vi "Find Center.vi"(5 "Position":i32, 7 "Tray Number":dbl format="%#_13g", 8 "Assembly Type":string, 9 "XYZTheta":dbl[](array[numeric]), 11 "Gantry In":refnum<k24>) -> (0 "Pedestal Height":dbl[](array[numeric]), 1 "XYZTheta Centers":dbl[][](array[numeric]), 3 "Gantry Out":refnum<k24>)   [LabVIEW 2021, in "Assembly Tray.lvclass"]
uses:
  Assembly Tray.lvclass
  Find Tray.ctl
  Controller/Camera/Machine Vision.ctl
  C:/Program Files (x86)/Aerotech/A3200/LabVIEW/2010/Bin/Aerotech.A3200.dll
  Program Files (x86)/Aerotech/A3200/LabVIEW/2010/Bin/Aerotech.A3200.dll
  Controller/Camera/Image processing.ctl
  Controller/Camera/Camera settings.ctl
  Controller/Camera/Material.ctl
  Controller/Camera/Camera.lvclass
  Controller/Motion/A3200/A3200.lvclass
  Controller/Motion/Motion.lvclass
panel:
  out "Current Z High Speed":dbl
  out "Current XY High Speed":dbl
  out "current Z low speed":dbl
  out "current XY speed":dbl
  in  "Z high":dbl=12.5
  in  "XY high":dbl=50.0
  in  "Z low":dbl=0.05
  in  "XY low":dbl=0.1
  out "Low Speed":bool
  out "X":bool
  out "Y":bool
  out "Z":bool
  out "High Speed":bool
  out "Move by":dbl[](array[numeric])
  in  "Autofiducial (Beta)":bool
  in  "Focus step size":dbl format="%#_13g"
  in  "number of focus steps":i32
  out "Average Strength":dbl
  in  "Focus":bool
  in  "Material":T1
  in  "Camera settings":T2={"Gamma"=1.6, "Gain"=0, "Sharpness"=0, "Contrast"=0.0, "Exposure"=0.0078125} {"Exposure" min=0.000244140625 max=0.5 scale=0.0002..0.5; "Contrast" min=0.0 max=1.0 scale=0.001..1.0; "Sharpness" min=0 max=2 step=1 scale=0.0..2.0; "Gain" min=0 max=100 step=1 scale=0.1..100.0; "Gamma" min=0.01 max=10.0 scale=0.01..10.0}
  in  "Image processing":T3={"Brightness"=128.0, "Contrast"=45.0, "Gamma"=1.0471123} {"Brightness" scale=0.0..400.0; "Contrast" scale=0.0..90.0; "Gamma" scale=0.005..5.0}
  in  "Override presets":bool
  out "Both fiducials recorded":bool
  in  "Machine Vision":T4
  out "Right Fiducial":dbl[](array[numeric]) format="%.6g"
  out "Left Fiducial":dbl[](array[numeric]) format="%.6g"
  out "Gantry":dbl[](array[numeric]) format="%.6g"
  out "Sum":dbl[](array[numeric]) format="%.6g"
  out "Camera":dbl[](array[numeric]) format="%.6g"
  in  "Carrier Tray":T5
  out "Image":T6(plugin-control)
  out "Center":dbl[](array[numeric]) format="%.6g"
  in  "Position Number":i16
  in  "Go to Center":bool
  in  "Calculate":bool
  in  "Record Bottom":bool
  in  "Record Top":bool
  in  "Go to Bottom Fiducial":bool
  in  "Go to Top Fiducial":bool
  in  "Joystick":bool
  in  "Stop":bool
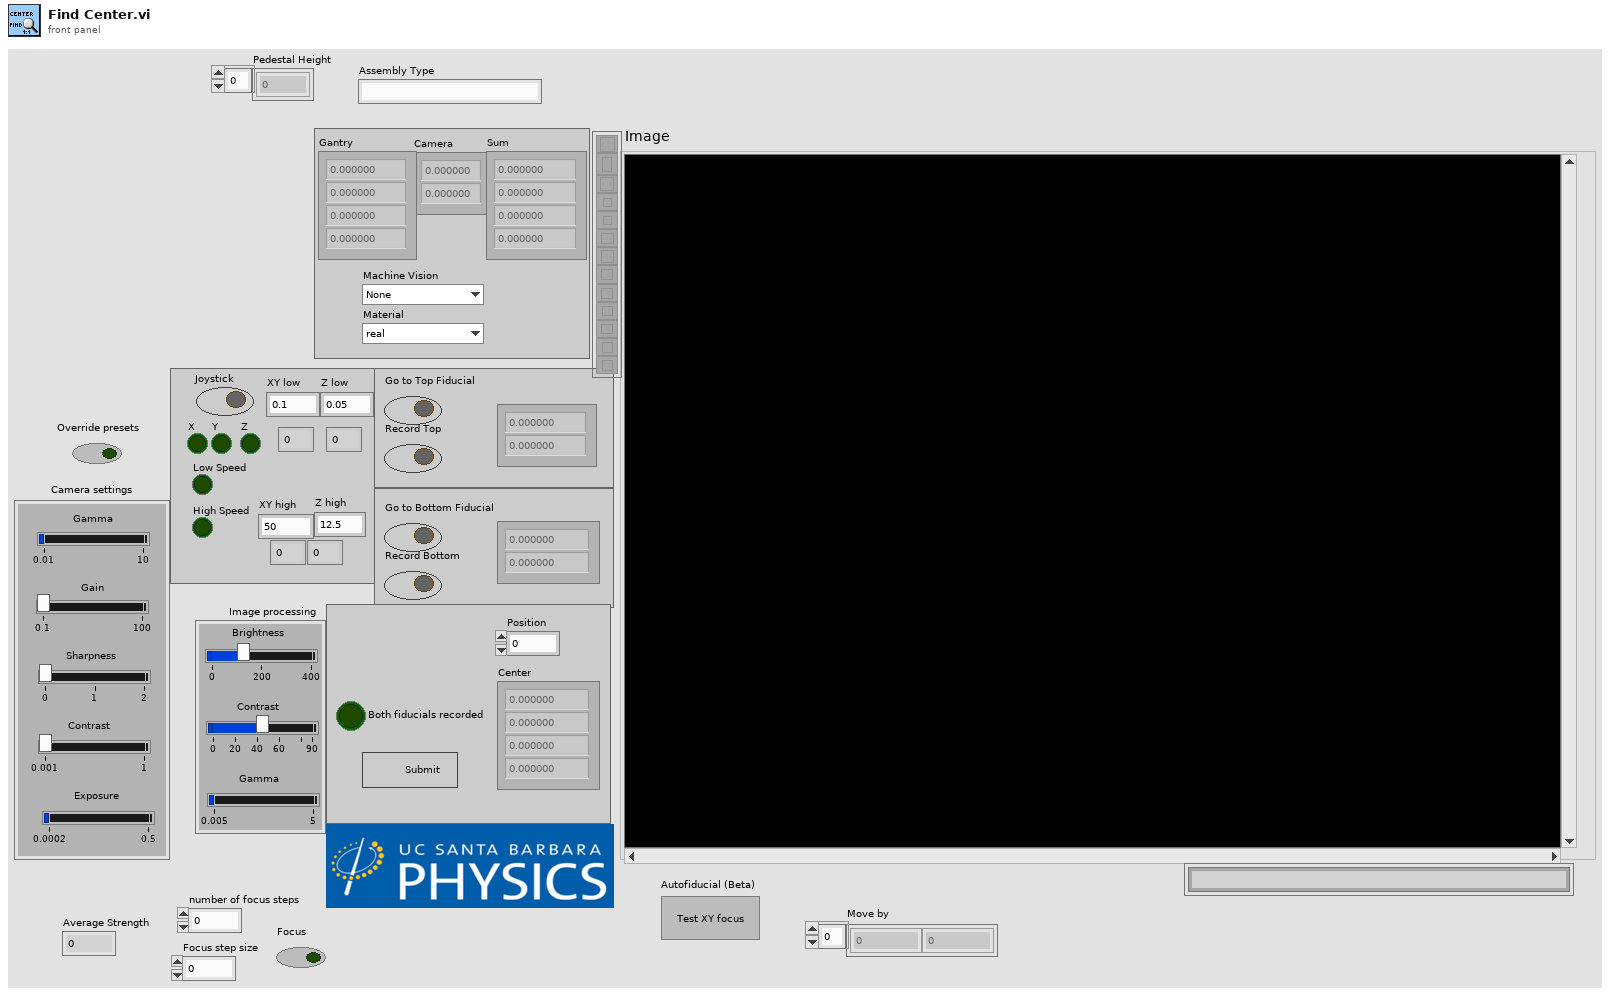
[diagram p1: front panel]
types:
  T1 = typedef "Camera.lvclass/Material.ctl" = enum16{"real", "dummy", "PETG"}
  T2 = typedef "Camera.lvclass/Camera settings.ctl" = cluster{"Gamma":dbl, "Gain":i64, "Sharpness":i64, "Contrast":dbl, "Exposure":dbl}
  T3 = typedef "Camera.lvclass/Image processing.ctl" = cluster{"Brightness":sgl, "Contrast":sgl, "Gamma":sgl}
  T4 = typedef "Camera.lvclass/Machine Vision.ctl" = enum16{"None", "Tray Fiducials", "Sensor Fiducials", "HPK Silicon", "Partial Hexaboard", "Partial Hexaboard Test", "100um dot", "Hexaboard", "Corner (TL, BR)", "Corner (BL, TR)", "V3 Sensor Cross", "V3 Sensor Circle", "test"}
  T5 = typedef "Assembly Tray.lvclass/Find Tray.ctl" = cluster{"Gantry Fiducials":dbl[], "Relative Coordinates":dbl[][], "Camera Fiducials":dbl[][], "XYZTheta Centers":dbl[][], "Workspace Center":dbl[], "Syringe Relative Coordinates":dbl[], "Gantry Region":dbl, "Fiducials":path, "New Fiducials":dbl[][], "Past Fiducials":dbl[][], "XYZTheta":dbl[], "Pedestal Height":dbl[]}
  T6 = typedef "IMAQ Image.ctl" = refnum<image>
  T7 = typedef "File Paths.ctl" = cluster{"Glue Pattern Folder":path, "Carrier Tray Folder":path, "Pick Up Tool Fixture Folder":path, "Components Folder":path, "Bellows Tool Offset.txt":path, "Pick Up Tool Offset.txt":path, "Dispense Tip Offset.txt":path, "Log Files":path, "Gantry Assembly Map.txt":path, "Syringe and offset map.txt":path, "Controllers Folder":path, "Local dbase config":path}
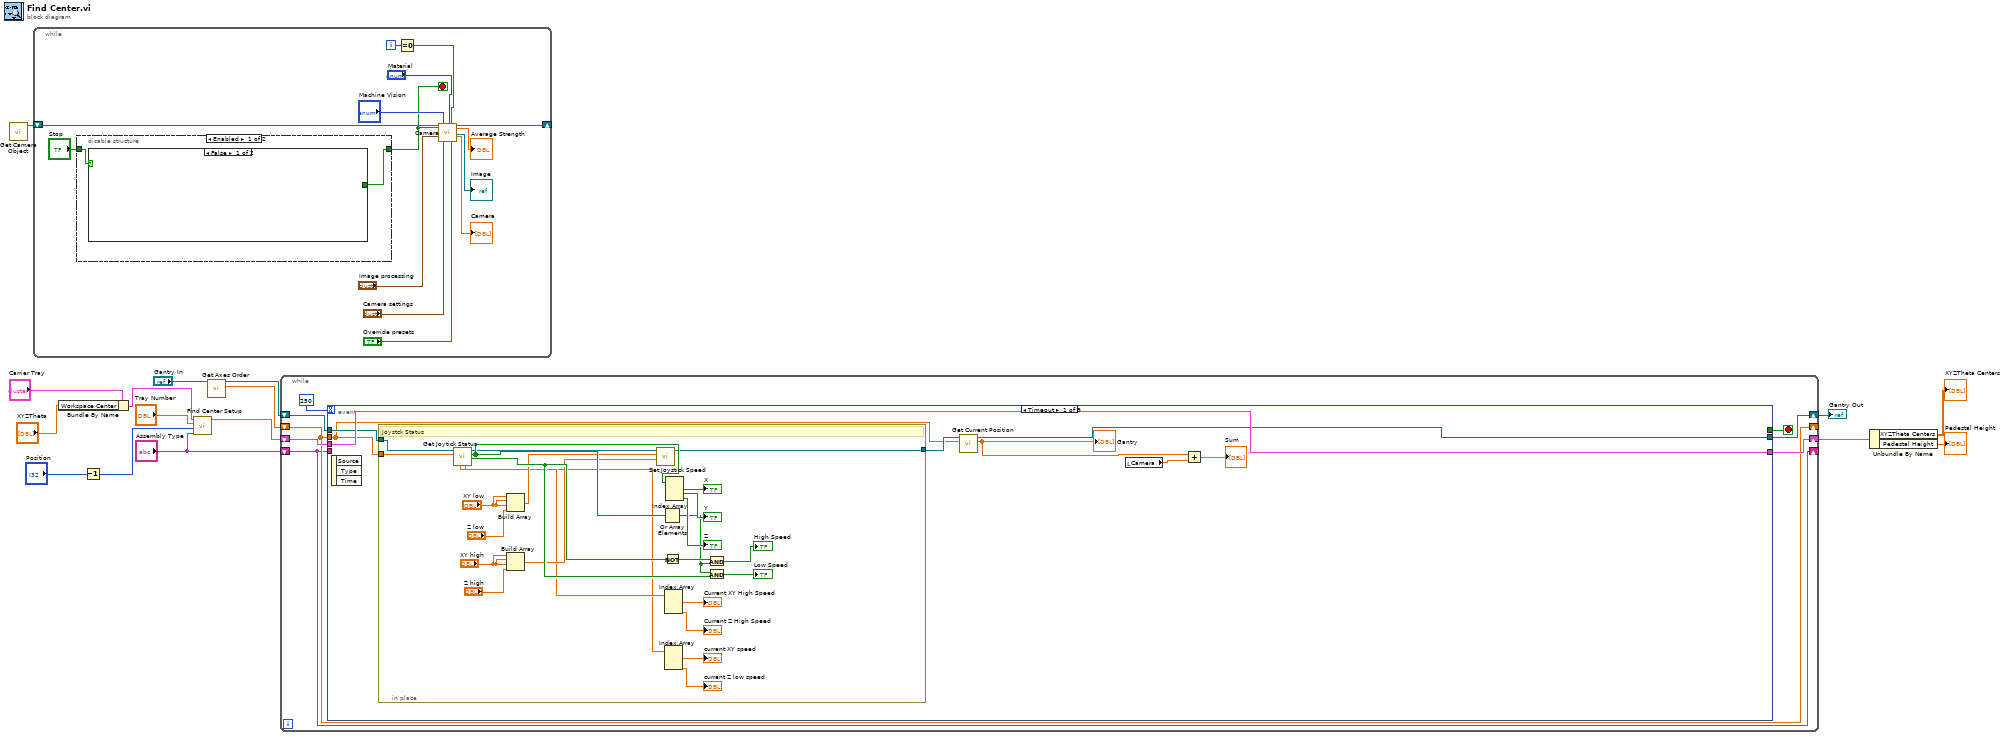
[diagram p0: block diagram]
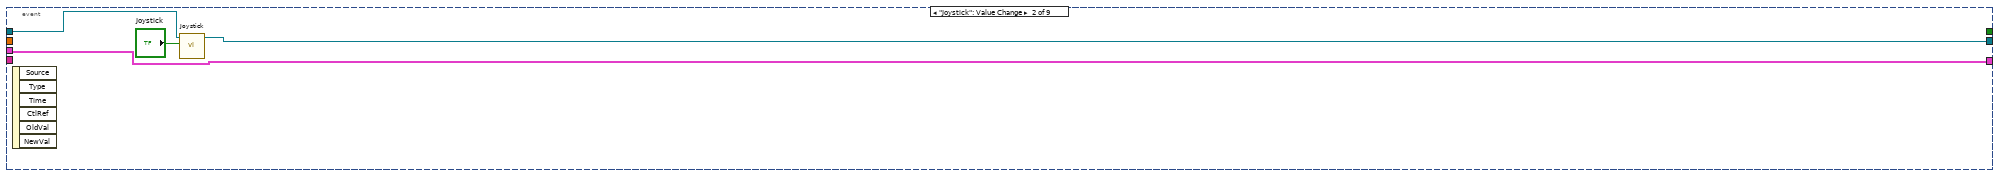
[diagram p2: hidden frame]
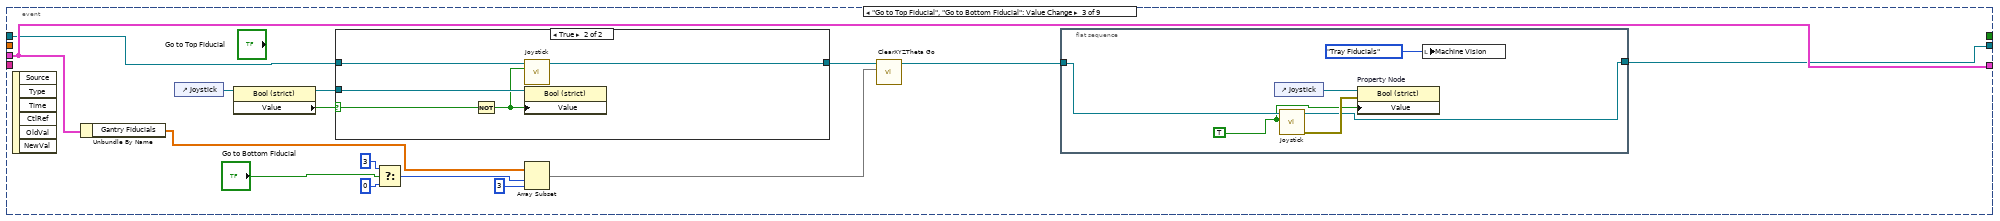
[diagram p3: hidden frame]
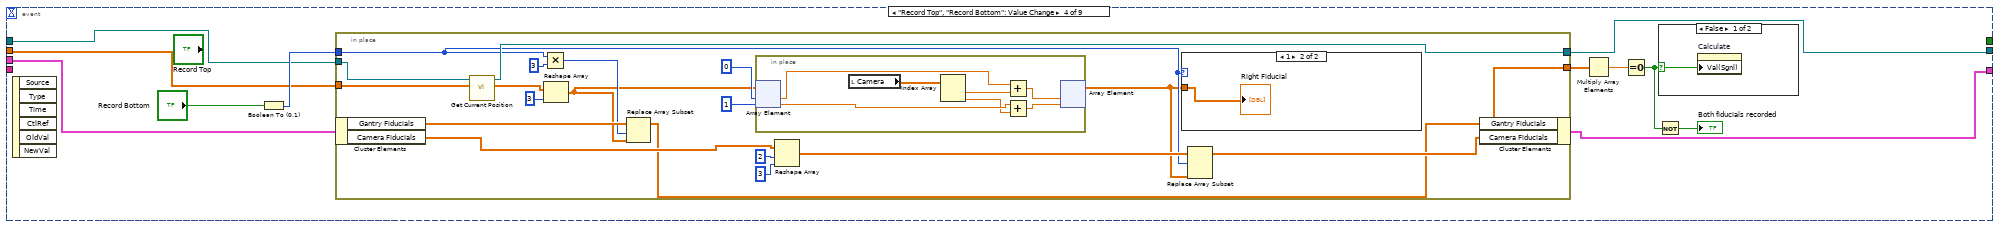
[diagram p5: hidden frame]
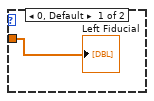
[diagram p7: hidden frame]
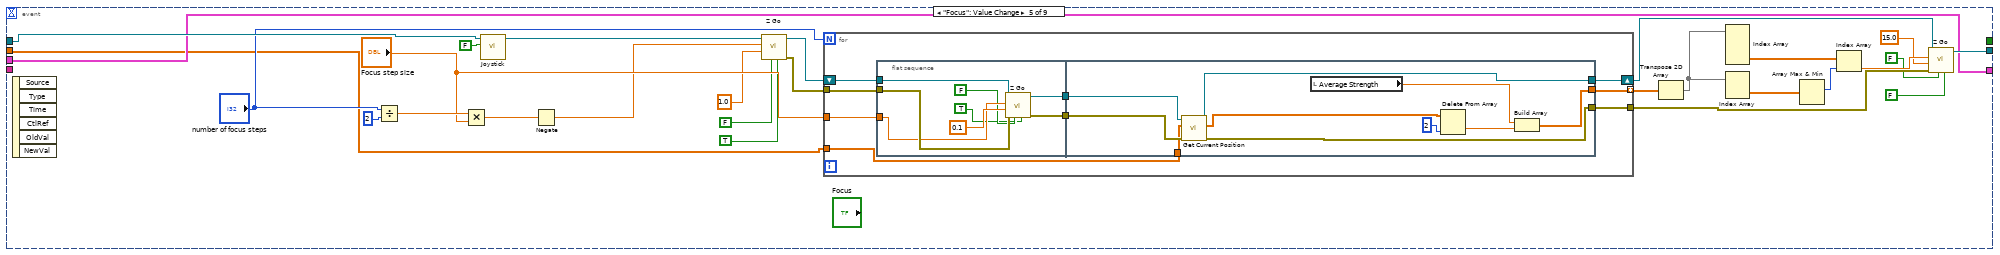
[diagram p8: hidden frame]
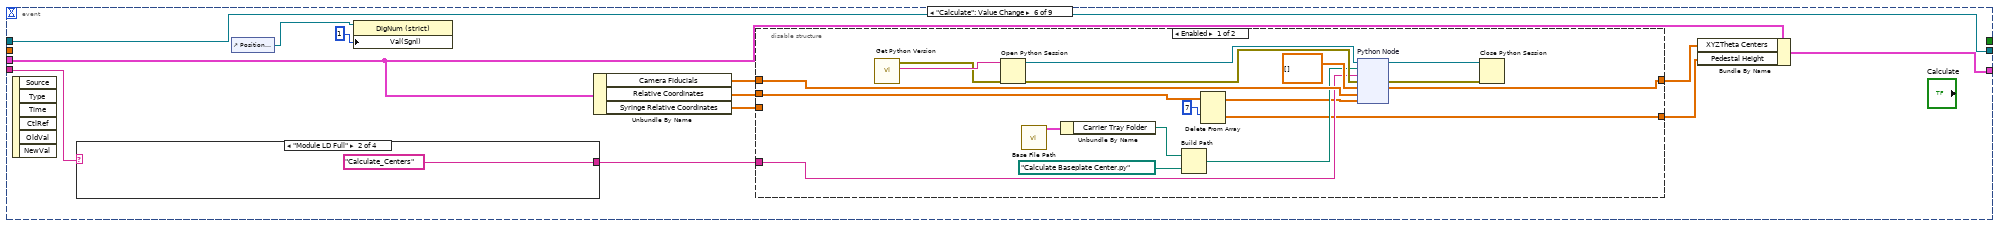
[diagram p9: hidden frame]
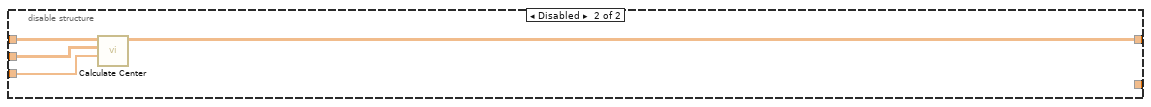
[diagram p10: hidden frame]
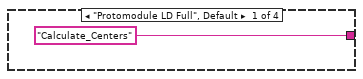
[diagram p11: hidden frame]
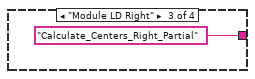
[diagram p12: hidden frame]
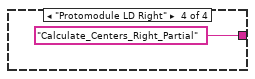
[diagram p13: hidden frame]
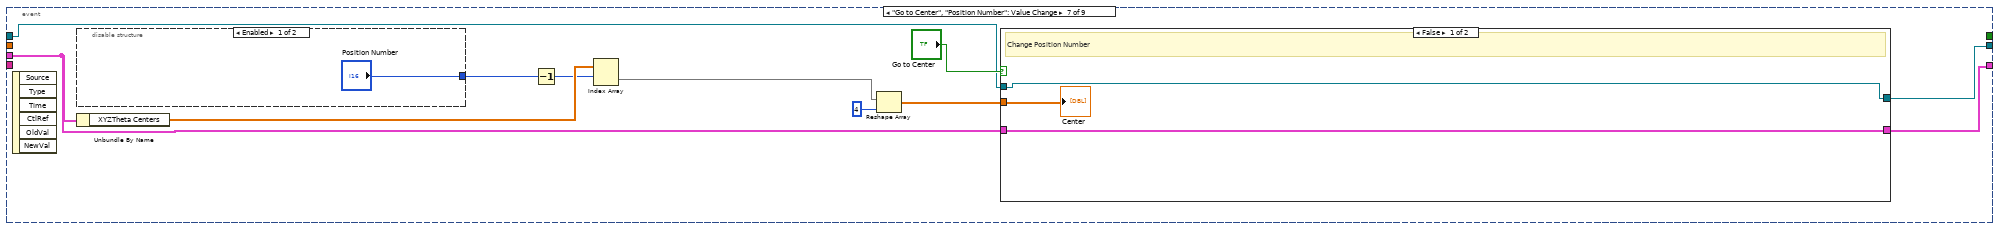
[diagram p14: hidden frame]
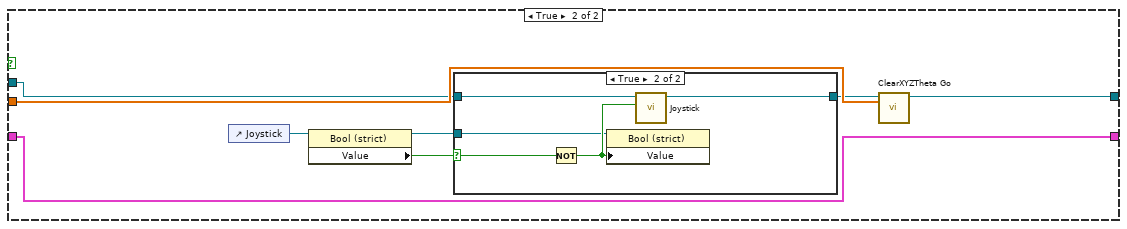
[diagram p16: hidden frame]
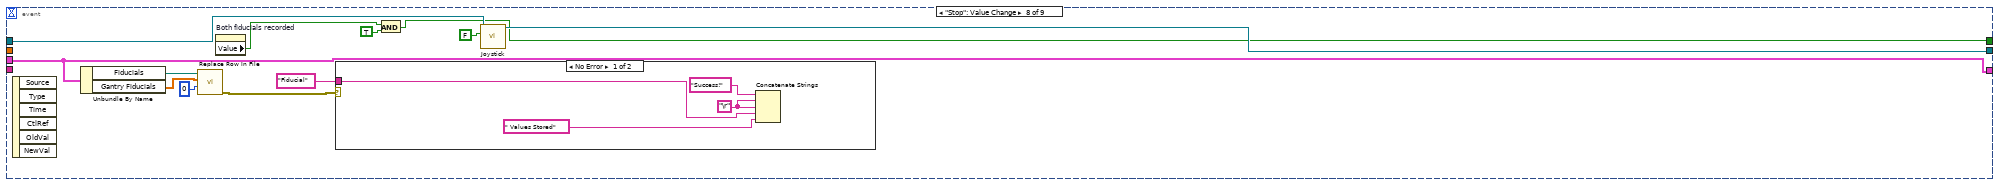
[diagram p18: hidden frame]
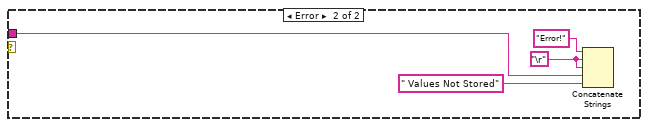
[diagram p19: hidden frame]
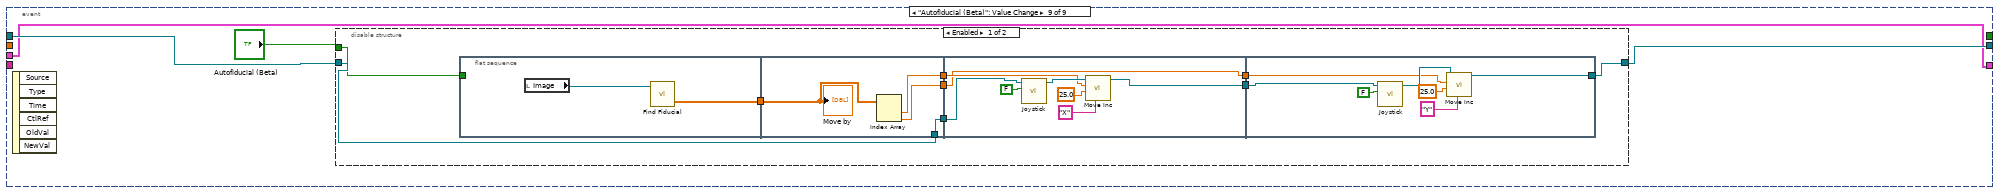
[diagram p20: hidden frame]
diagram:
  n1 = call "Get Camera Object.vi"() -> ("Camera out"=w9:refnum<class "Camera.lvclass">)  [unwired: 10 in, 1 out]
  n2 = while {
    shift-right: [w26] -> _
    shift-left: w9 -> [w30]
    i -> [w20]
    stop <- w25 stop-if-true
    n3 = disable-structure shown="Enabled" {
      disable-tunnel: [w31 w38] -> w25
      disable-tunnel: "Stop" -> [w32 w38]
      frame Enabled {
        n4 = case shown="False" w32 {
          tunnel: [_ w33] -> w31
          frame False {
          }
          frame True {
            n5 = property on="Both fiducials recorded" class="Bool (strict)"() -> ("Value"=w34:bool)  [unwired: 2 in, 2 out]
            n6 = case shown="False" w34 {
              tunnel: [_ TRUE] -> w33
              frame False {
                n7 = One Button Dialog(message="Atleast one fiducial not recorded!") -> ()  [unwired: 1 in, 1 out]
              }
              frame True {
                n8 = property on="Both fiducials recorded" class="Bool (strict)"("Val(Sgnl)"=FALSE) -> ()  [unwired: 2 in, 2 out]
              }
            }
          }
        }
      }
      frame Disabled {
      }
    }
    n9 = Equal To 0?(x=w20) -> (x = 0?=w19:bool)
    n10 = call "Camera.vi"("Camera in"=w30, "Stop"=w25, "BCG Image Processing"="Image processing", "Machine Vision"="Machine Vision", "Camera settings"="Camera settings", "Material"="Material", "Loop 0"=w19, "Override presets"="Override presets") -> ("Camera out"=w26:refnum<class "Camera.lvclass">, "Average Strength"=→"Average Strength":dbl, "Image"=→"Image":T6, "Camera"=→"Camera":dbl[])  [unwired: 5 in, 3 out]
  }
  n11 = Bundle By Name(cluster="Carrier Tray", "Workspace Center"="XYZTheta") -> (w13:T5)
  n12 = Decrement(x="Position") -> (x-1=w7:i32)
  n13 = call "Find Center Setup.vi"("Carrier Tray"=w13, "Tray Number"="Tray Number", "Position"=w7, "Assembly Type"="Assembly Type") -> ("Assembly Tray Out"=w16:T5)  [unwired: 6 in]
  n14 = call "Get Axes Order.vi"("Gantry In"="Gantry In") -> ("Axes Order"=w3:dbl[], "Gantry Out"=w4:refnum<k24>)  [unwired: 8 in, 1 out]
  n15 = while {
    shift-right: [w45] -> w15
    shift-left: w16 -> [w46]
    shift-right: [w41] -> w8
    shift-left: w4 -> [w42]
    shift-right: [w40] -> _
    shift-left: w3 -> [w40]
    shift-right: [w39] -> _
    shift-left: "Assembly Type" -> [w39]
    stop <- w44 stop-if-true
    n16 = event shown="[0] Timeout" {
      selector: _ -> [_ _ _ _ _ _ _ _ _]
      dyn-events: _ -> [_ _ _ _ _ _ _ _ _]
      timeout: 250 -> [_ _ _ _ _ _ _ _ _]
      tunnel: [w52 w83 w98 w121 w163 w209 w253 w280 w293] -> w45
      tunnel: w46 -> [w52 w83 w98 w116 w163 w210 w254 w280 w293]
      tunnel: [_ _ _ _ _ _ _ w275 _] -> w44
      tunnel: w42 -> [w49 w82 w90 w115 w165 w215 w251 w281 w295]
      tunnel: [w50 w80 w85 w114 w164 w215 w248 w276 w296] -> w41
      tunnel: w39 -> [_ _ _ _ _ w211 _ _ _]
      tunnel: w40 -> [w47 _ _ w111 w151 _ _ _ _]
      event Timeout {
        n17 = event-data() -> ()  [unwired: 1 in, 3 out]
        n18 = in-place {
          in-place-border: w49 -> [w79]
          in-place-border: [w59] -> w48
          in-place-border: w47 -> [w78]
          # "Joystck Status"
          n19 = call "Get Joytick Status.vi"("Axes Order"=w78, "Gantry In"=w79) -> ("JoystickLowSpeedActive"=w72:bool, "Joystick Status"=w74:bool[], "Gantry Out"=w60:refnum<k24>, "High Speeds"=w56:dbl[], "Low Speeds"=w55:dbl[])  [unwired: 4 in, 1 out]
          n20 = Build Array("XY low", "XY low", "XY low", "Z low") -> (w58:dbl[])
          n21 = Build Array("XY high", "XY high", "XY high", "Z high") -> (w57:dbl[])
          n22 = call "Set Joystick Speed.vi"("High Speed Inputs"=w57, "Low Speed Inputs"=w58, "Gantry"=w60) -> ("Controller Out"=w59:refnum<k24>)  [unwired: 7 in, 1 out]
          n23 = Or Array Elements(Boolean array=w74) -> (logical OR=w70:bool)
          n24 = Not(x=w72) -> (.not. x?=w71:bool)
          n25 = Index Array(array=w56) -> (element #1=→"Current XY High Speed":dbl, element #3=→"Current Z High Speed":dbl)  [unwired: 3 in, 1 out]
          n26 = Index Array(array=w55) -> (element #1=→"current XY speed":dbl, element #3=→"current Z low speed":dbl)  [unwired: 3 in, 1 out]
          n27 = Index Array(array=w74) -> (element #1=→"X":bool, element #2=→"Y":bool, element #3=→"Z":bool)  [unwired: 3 in]
          n28 = And(x=w71, y=w70) -> (x .and. y?=→"High Speed":bool)
          n29 = And(x=w70, y=w72) -> (x .and. y?=→"Low Speed":bool)
        }
        n30 = call "Get Current Position.vi"("Axes Order"=w47, "Gantry In"=w48) -> ("XYZTheta Out"=w51:dbl[], "Gantry Out"=w50:refnum<k24>)  [unwired: 7 in, 1 out]
        "Gantry" <- w51
        n31 = local read "Camera"() -> (w54:dbl[])
        n32 = Add(x=w51, y=w54) -> (x+y=→"Sum":dbl[])
      }
      event "Joystick": Value Change {
        n33 = event-data() -> ()  [unwired: 1 in, 6 out]
        n34 = call "Joystick.vi"("Joystick"="Joystick", "Gantry In"=w82) -> ("Gantry Out"=w80:refnum<k24>)  [unwired: 8 in, 1 out]
      }
      event "Go to Top Fiducial", "Go to Bottom Fiducial": Value Change {
        n35 = event-data() -> ()  [unwired: 1 in, 6 out]
        n36 = Unbundle By Name "Unbundle By Name"(w98) -> ("Gantry Fiducials"=w87:dbl[])
        n37 = control-ref of="Joystick"() -> (w97:refnum<vi>)
        n38 = property class="Bool (strict)"(reference=w97) -> (reference out=w88:refnum<vi>, "Value"=w91:bool)  [unwired: 1 in, 1 out]
        n39 = case shown="True" w91 {
          selector: w91 -> [_ w110]
          tunnel: w90 -> [w105 w108]
          tunnel: [w105 w107] -> w89
          tunnel: w88 -> [_ w109]
          frame False {
          }
          frame True {
            n40 = Not(x=w110) -> (.not. x?=w106:bool)
            n41 = call "Joystick.vi"("Joystick"=w106, "Gantry In"=w108) -> ("Gantry Out"=w107:refnum<k24>)  [unwired: 8 in, 1 out]
            n42 = property class="Bool (strict)"(reference=w109, "Value"=w106) -> ()  [unwired: 1 in, 2 out]
          }
        }
        n43 = Select(t=3, s="Go to Bottom Fiducial", f=0) -> (s? t:f=w95:i32)
        n44 = Array Subset "Array Subset"(array=w87, index=w95, length=3) -> (w86:dbl[])
        n45 = call "ClearXYZTheta Go.vi"("XYZTheta In"=w86, "Gantry In"=w89) -> ("Gantry Out"=w84:refnum<k24>)  [unwired: 7 in, 2 out]
        n46 = flat-sequence {
          tunnel: w84 -> [w104]
          tunnel: [w101] -> w85
          frame #0 {
            w100 = TRUE
            n47 = control-ref of="Joystick"() -> (w103:refnum<vi>)
            n48 = call "Joystick.vi"("Joystick"=w100, "Gantry In"=w104) -> ("error out"=w102:errorcluster, "Gantry Out"=w101:refnum<k24>)  [unwired: 8 in]
            n49 = property on="Property Node" class="Bool (strict)"(reference=w103, error in=w102, "Value"=w100) -> ()  [unwired: 2 out]
            n50 = local write "Machine Vision"(Machine_Vision."Tray Fiducials" ("Machine Vision")) -> ()
          }
        }
      }
      event "Record Top", "Record Bottom": Value Change {
        n51 = event-data() -> ()  [unwired: 1 in, 6 out]
        n52 = Boolean To (0,1)(Boolean="Record Bottom") -> (0, 1=w118:i16)
        n53 = in-place {
          in-place-border: [w135] -> w119
          in-place-border: w118 -> [w128]
          in-place-border: w115 -> [w130]
          in-place-border: [w129] -> w114
          in-place-border: w111 -> [w123]
          n54 = in-place-cluster #1(w116) -> ("Gantry Fiducials"=w132:dbl[], "Camera Fiducials"=w139:dbl[][])
          n55 = call "Get Current Position.vi"("Axes Order"=w123, "Gantry In"=w130) -> ("XYZTheta Out"=w133:dbl[], "Gantry Out"=w129:refnum<k24>)  [unwired: 7 in, 1 out]
          n56 = Multiply(x=w128, y=i16 3) -> (x*y=w126:i16)
          n57 = Reshape Array(w133, 3 ("dimension size")) -> (w125:dbl[])
          n58 = Replace Array Subset(array=w132, new element=w125, index=w126) -> (w131:dbl[])
          n59 = in-place {
            n60 = in-place-array #2(w125, 0, 1) -> (w147:dbl, w145:dbl)
            n61 = local read "Camera"() -> (w148:dbl[])
            n62 = Index Array(array=w148) -> (element #1=w146:dbl, element #2=w144:dbl)  [unwired: 2 in]
            n63 = Add(x=w147, y=w146) -> (x+y=w142:dbl)
            n64 = Add(x=w145, y=w144) -> (x+y=w143:dbl)
            n65 = in-place-array #2(w142, w143) -> (w124:dbl[])  [unwired: 2 out]
          }
          n66 = Reshape Array(w139, 2 ("length"), 3 ("dimension size")) -> (w138:dbl[][])
          n67 = case shown="1" w128 {
            tunnel: w124 -> [w149 w150]
            frame 0, Default {
              "Left Fiducial" <- w149
            }
            frame 1 {
              "Right Fiducial" <- w150
            }
          }
          n68 = Replace Array Subset(array=w138, new element=w124, index (row)=w128) -> (w135:dbl[][])  [unwired: 1 in]
          n69 = in-place-cluster #1("Gantry Fiducials"=w131, "Camera Fiducials"=w135) -> (w121:T5)
        }
        n70 = Multiply Array Elements(1:w119) -> (0:w120:dbl)
        n71 = Equal To 0?(x=w120) -> (x = 0?=w113:bool)
        n72 = Not(x=w113) -> (.not. x?=→"Both fiducials recorded":bool)
        n73 = case shown="False" w113 {
          selector: w113 -> [w122 _]
          frame False {
            n74 = property on="Calculate" class="Bool (strict)"("Val(Sgnl)"=w122) -> ()  [unwired: 2 in, 2 out]
          }
          frame True {
          }
        }
      }
      event "Focus": Value Change {
        n75 = event-data() -> ()  [unwired: 1 in, 6 out]
        n76 = Divide(x="number of focus steps", y=2) -> (x/y=w167:dbl)
        n77 = Multiply(x=w167, y="Focus step size") -> (x*y=w166:dbl)
        n78 = call "Joystick.vi"("Joystick"=FALSE, "Gantry In"=w165) -> ("Gantry Out"=w159:refnum<k24>)  [unwired: 8 in, 1 out]
        n79 = Negate(x=w166) -> (-x=w157:dbl)
        n80 = call "Z Go.vi"("Increment"=TRUE, "Return Immediately"=FALSE ("Increment"), "Speed In"=1.0 ("Speed"), "Position In"=w157, "Gantry In"=w159) -> ("error out"=w154:errorcluster, "Gantry Out"=w158:refnum<k24>)  [unwired: 3 in, 2 out]
        n81 = for {
          N: "number of focus steps" -> [_]
          tunnel: [w184] -> w177 mode=indexing
          tunnel: w154 -> [w183]
          tunnel: [w181] -> w170
          shift-right: [w185] -> w171
          shift-left: w158 -> [w187]
          tunnel: "Focus step size" -> [w180]
          tunnel: w151 -> [w179]
          n82 = flat-sequence {
            tunnel: w187 -> [w195]
            tunnel: [w194] -> w186
            tunnel: w183 -> [w192]
            tunnel: [w193] -> w182
            tunnel: w180 -> [w190]
            tunnel: w186 -> [w205]
            tunnel: [w204] -> w185
            tunnel: [w203] -> w184
            tunnel: w182 -> [w199]
            tunnel: [w198] -> w181
            tunnel: w179 -> [w196]
            frame #0 {
              n83 = call "Z Go.vi"("Increment"=TRUE, "Return Immediately"=FALSE ("Increment"), "error in (no error)"=w192, "Speed In"=0.1 ("Speed"), "Position In"=w190, "Gantry In"=w195) -> ("error out"=w193:errorcluster, "Gantry Out"=w194:refnum<k24>)  [unwired: 2 in, 2 out]
            }
            frame #1 {
              n84 = call "Get Current Position.vi"("error in (no error)"=w199, "Axes Order"=w196, "Gantry In"=w205) -> ("error out"=w198:errorcluster, "XYZTheta Out"=w202:dbl[], "Gantry Out"=w204:refnum<k24>)  [unwired: 6 in]
              n85 = local read "Average Strength"() -> (w197:dbl)
              n86 = Delete From Array(array=w202, index=2) -> (deleted portion=w200:dbl)  [unwired: 1 in, 1 out]
              n87 = Build Array(w197, w200) -> (w203:dbl[])
            }
          }
        }
        n88 = Transpose 2D Array(2D array=w177) -> (transposed array=w176:dbl[][])
        n89 = Index Array(array=w176) -> (element #2=w175:dbl[])  [unwired: 4 in, 1 out]
        n90 = Index Array(array=w176) -> (element=w178:dbl[])  [unwired: 2 in]
        n91 = Array Max & Min(array=w178) -> (max index (indices)=w174:i32)  [unwired: 3 out]
        n92 = Index Array(array=w175, index=w174) -> (element=w173:dbl)
        n93 = call "Z Go.vi"("Increment"=FALSE, "Return Immediately"=FALSE ("Increment"), "error in (no error)"=w170, "Speed In"=15.0 ("Speed"), "Position In"=w173, "Gantry In"=w171) -> ("Gantry Out"=w164:refnum<k24>)  [unwired: 2 in, 3 out]
      }
      event "Calculate": Value Change {
        n94 = event-data() -> ()  [unwired: 1 in, 6 out]
        n95 = case shown="\"Module LD Full\"" w211 {
          tunnel: ["Calculate_Centers" ("function name") "Calculate_Centers" ("function name") "Calculate_Centers_Right_Partial" ("function name") "Calculate_Centers_Right_Partial" ("function name")] -> w208
          frame "Protomodule LD Full", Default {
          }
          frame "Module LD Full" {
          }
          frame "Module LD Right" {
          }
          frame "Protomodule LD Right" {
          }
        }
        n96 = control-ref of="Position Number"() -> (w217:refnum<vi>)
        n97 = property class="DigNum (strict)"(reference=w217, "Val(Sgnl)"=i16 1 ("Value (Signaling)")) -> ()  [unwired: 1 in, 2 out]
        n98 = Unbundle By Name "Unbundle By Name"(w210) -> ("Camera Fiducials"=w212:dbl[][], "Relative Coordinates"=w213:dbl[][], "Syringe Relative Coordinates"=w214:dbl[])
        n99 = disable-structure shown="Enabled" {
          disable-tunnel: w212 -> [w230 w238]
          disable-tunnel: w213 -> [w221 w237]
          disable-tunnel: w214 -> [_ w236]
          disable-tunnel: [w225 w239] -> w207
          disable-tunnel: w208 -> [w224 _]
          disable-tunnel: [w218 _] -> w206
          frame Enabled {
            n100 = call "Get Python Version.vi"() -> ("Python Version"=w223:string, "error out"=w222:errorcluster)  [unwired: 10 in]
            n101 = Open Python Session(python version=w223, 3:w222) -> (session out=w235:refnum<k35>, error out=w233:errorcluster)  [unwired: 1 in]
            n102 = call "Base File Path.vi"() -> ("Paths Out"=w231:T7)  [unwired: 11 in]
            n103 = Unbundle By Name(w231) -> ("Carrier Tray Folder"=w228:path)
            n104 = Build Path(base path=w228, name or relative path=path "Calculate Baseplate Center.py") -> (appended path=w227:path)
            n105 = Delete From Array(array=w221, index (row)=7) -> (deleted portion=w218:dbl[], array with subset deleted=w219:dbl[][])  [unwired: 2 in]
            n106 = node "Python Node"(w235, w227, w224, w233, dbl[][] [], w230, w219) -> (w234:refnum<k35>, w232:errorcluster, w225:dbl[][])  [unwired: 2 in, 2 out]
            n107 = Close Python Session(session in=w234, error in=w232) -> ()  [unwired: 1 out]
          }
          frame Disabled {
            n108 = call "Calculate Center.vi"("Syringe Coordinates"=w236, "Relative Coordinates"=w237, "Fiducial Measurements"=w238) -> ("XYZTheta Centers"=w239:dbl[][])  [unwired: 8 in]
          }
        }
        n109 = Bundle By Name(cluster=w210, "XYZTheta Centers"=w207, "Pedestal Height"=w206) -> (w209:T5)
      }
      event "Go to Center", "Position Number": Value Change {
        n110 = event-data() -> ()  [unwired: 1 in, 6 out]
        n111 = disable-structure shown="Enabled" {
          disable-tunnel: ["Position Number" _] -> w245
          frame Enabled {
          }
          frame Disabled {
          }
        }
        n112 = Unbundle By Name(w254) -> ("XYZTheta Centers"=w247:dbl[][])
        n113 = Decrement(x=w245) -> (x-1=w246:i16)
        n114 = Index Array "Index Array"(array=w247, index (row)=w246) -> (element=w249:dbl[])  [unwired: 1 in]
        n115 = Reshape Array "Reshape Array"(w249, u32 4) -> (w244:dbl[])
        n116 = case shown="False" "Go to Center" {
          tunnel: w244 -> [w256 w264]
          tunnel: w254 -> [w258 w266]
          tunnel: [w258 w266] -> w253
          tunnel: w251 -> [w257 w260]
          tunnel: [w257 w265] -> w248
          frame False {
            # "Change Position Number"
            "Center" <- w256
          }
          frame True {
            n117 = control-ref of="Joystick"() -> (w263:refnum<vi>)
            n118 = property class="Bool (strict)"(reference=w263) -> (reference out=w261:refnum<vi>, "Value"=w262:bool)  [unwired: 1 in, 1 out]
            n119 = case shown="True" w262 {
              selector: w262 -> [_ w272]
              tunnel: w260 -> [w267 w271]
              tunnel: [w267 w270] -> w259
              tunnel: w261 -> [_ w268]
              frame False {
              }
              frame True {
                n120 = Not(x=w272) -> (.not. x?=w269:bool)
                n121 = property class="Bool (strict)"(reference=w268, "Value"=w269) -> ()  [unwired: 1 in, 2 out]
                n122 = call "Joystick.vi"("Joystick"=w269, "Gantry In"=w271) -> ("Gantry Out"=w270:refnum<k24>)  [unwired: 8 in, 1 out]
              }
            }
            n123 = call "ClearXYZTheta Go.vi"("XYZTheta In"=w264, "Gantry In"=w259) -> ("Gantry Out"=w265:refnum<k24>)  [unwired: 7 in, 2 out]
          }
        }
      }
      event "Stop": Value Change {
        n124 = event-data() -> ()  [unwired: 1 in, 6 out]
        n125 = Unbundle By Name(w280) -> ("Fiducials"=w278:path, "Gantry Fiducials"=w279:dbl[])
        n126 = call "Replace Row In File.vi"("Index"=0, "Insert Array"=w279, "Path"=w278) -> ("error out"=w284:errorcluster)  [unwired: 8 in]
        n127 = property on="Both fiducials recorded" class="Bool (strict)"() -> ("Value"=w273:bool)  [unwired: 2 in, 2 out]
        n128 = case shown="No Error" w284 {
          tunnel: "Fiducial" -> [w285 w292]
          frame No Error {
            w286 = "\r"
            n129 = Concatenate Strings("Success!", w286, w286, w285, " Values Stored") -> ()  [unwired: 1 out]
          }
          frame Error {
            w289 = "\r"
            n130 = Concatenate Strings("Error!", w289, w289, w292, " Values Not Stored") -> ()  [unwired: 1 out]
          }
        }
        n131 = And(x=w273, y=TRUE) -> (x .and. y?=w275:bool)
        n132 = call "Joystick.vi"("Joystick"=FALSE, "Gantry In"=w281) -> ("Gantry Out"=w276:refnum<k24>)  [unwired: 8 in, 1 out]
      }
      event "Autofiducial (Beta)": Value Change {
        n133 = event-data() -> ()  [unwired: 1 in, 6 out]
        n134 = disable-structure shown="Enabled" {
          disable-tunnel: [w300 w327] -> w296
          disable-tunnel: w295 -> [w299 w327]
          disable-tunnel: "Autofiducial (Beta)" -> [w298 _]
          frame Enabled {
            n135 = flat-sequence {
              tunnel: w298 -> [_]
              tunnel: [w306] -> w297
              tunnel: w299 -> [w311]
              tunnel: [w311] -> w305
              tunnel: [w310] -> w304
              tunnel: [w309] -> w303
              tunnel: w297 -> [w308]
              tunnel: w305 -> [w315]
              tunnel: [w314] -> w302
              tunnel: w304 -> [w313]
              tunnel: [w312] -> w301
              tunnel: w303 -> [w312]
              tunnel: [w321] -> w300
              tunnel: w302 -> [w322]
              tunnel: w301 -> [w320]
              frame #0 {
                n136 = local read "Image"() -> (w307:T6)
                n137 = call "Find Fiducial.vi"("Image"=w307) -> ("Move by (mm)"=w306:dbl[])  [unwired: 3 in]
              }
              frame #1 {
                n138 = Index Array(array=w308) -> (element #1=w310:dbl, element #2=w309:dbl)  [unwired: 2 in]
                "Move by" <- w308
              }
              frame #2 {
                n139 = call "Joystick.vi"("Joystick"=FALSE, "Gantry In"=w315) -> ("Gantry Out"=w316:refnum<k24>)  [unwired: 8 in, 1 out]
                n140 = call "Move Inc.vi"("Axis"="X", "Speed"=25.0, "Distance"=w313, "Gantry In"=w316) -> ("Gantry Out"=w314:refnum<k24>)  [unwired: 6 in, 1 out]
              }
              frame #3 {
                n141 = call "Joystick.vi"("Joystick"=FALSE, "Gantry In"=w322) -> ("Gantry Out"=w323:refnum<k24>)  [unwired: 8 in, 1 out]
                n142 = call "Move Inc.vi"("Axis"="Y", "Speed"=25.0, "Distance"=w320, "Gantry In"=w323) -> ("Gantry Out"=w321:refnum<k24>)  [unwired: 6 in, 1 out]
              }
            }
          }
          frame Disabled {
          }
        }
      }
    }
  }
  "Gantry Out" <- w8
  n143 = Unbundle By Name(w15) -> ("XYZTheta Centers"=→"XYZTheta Centers":dbl[][], "Pedestal Height"=→"Pedestal Height":dbl[])
